vi "RemoteVI VI Server Request.vi"(0 "put?":bool, 1 "hWnd":u64, 2 "address":string, 11 "error in":errorcluster) -> (4 "stored?":bool, 5 "address out":string, 15 "error out":errorcluster)   [LabVIEW 2020, in "RemoteVI.lvlib"]
doc: "Hands the VI Server address of a window share from RemoteVI Launch Share.vi to the share's server loop (RemoteVI Server Setup.vi, which connects in the loop so the loop owns the references) - a functional global with one slot (a Feedback Node outside any loop); Launch Share waits until the loop has started, so one slot is enough. put? TRUE stores address for hWnd; FALSE takes the address stored for hWnd (address out; empty and stored? FALSE when none was stored for this hWnd). address: empty = find out from the application's INI file (server.tcp.enabled, server.tcp.port), off = window only, host:port = that VI Server."
uses:
  RemoteVI.lvlib
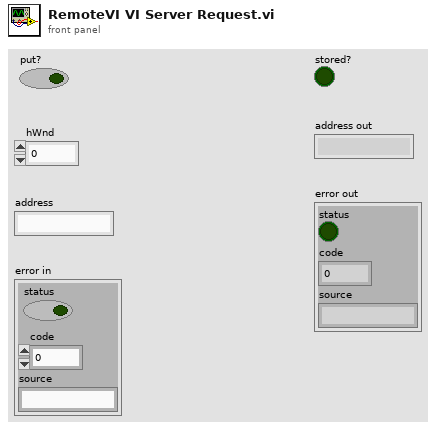
[diagram p1: front panel]
types:
  T1 = cluster{"valid":bool, "hWnd":u64, "address":string}
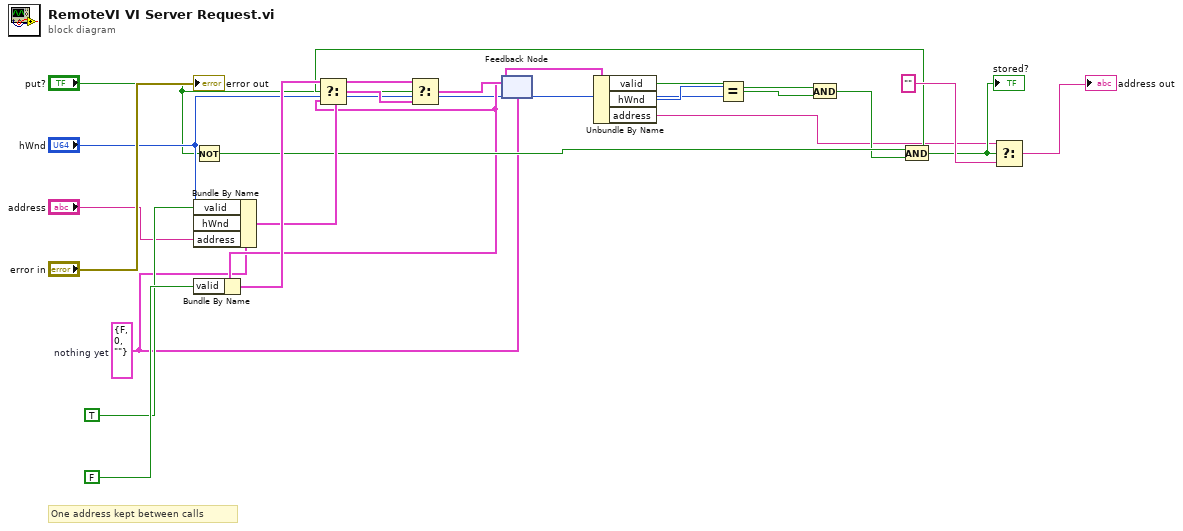
[diagram p0: block diagram]
diagram:
  w5 = T1 {"valid"=FALSE, "hWnd"=0, "address"=""}  # nothing yet
  # "One address kept between calls"
  n1 = Not(x="put?") -> (.not. x?=w13:bool)
  n2 = Bundle By Name(cluster=w5, "valid"=TRUE, "hWnd"="hWnd", "address"="address") -> (w17:T1)
  n3 = feedback #1(w5) -> (w6:T1)
  n4 = Bundle By Name(cluster=w6, "valid"=FALSE) -> (w18:T1)
  n5 = Unbundle By Name(w6) -> ("valid"=w8:bool, "hWnd"=w9:u64, "address"=w10:string)
  n6 = Equal?(x=w9, y="hWnd") -> (x = y?=w11:bool)
  n7 = And(x=w8, y=w11) -> (x .and. y?=w12:bool)
  n8 = And(x=w13, y=w12) -> (x .and. y?=w14:bool)
  "stored?" <- w14
  n9 = Select(t=w18, s=w14, f=w6) -> (s? t:f=w19:T1)
  n10 = Select(t=w17, s="put?", f=w19) -> (s? t:f=w7:T1)
  n11 = feedback-in #1(w7) -> ()
  n12 = Select(t=w10, s=w14, f="") -> (s? t:f=→"address out":string)
  "error out" <- "error in"
